vi "Test_C_WS_to_CAN_to_WS.vi"() -> ()   [LabVIEW 2021]
uses:
  CANsub_C.lvlib
  codec_vis/CANsub_Codec.lvlib
  common/Typedefs/Bytes.ctl
  common/CANsub_Common.lvlib
  common/Typedefs/CAN_Frame.ctl
  C_Decode_Result.ctl
panel:
  out "error out":errorcluster
  out "ping payload":u8[](array[numeric]) format="%.0x"
  out "C_Decode_Result":T1={"n frames"=1, "peer close"=FALSE, "ping len"=-1, "crc errors"=0, "decode errors"=0}
  out "frames":T2[](array[typedef])=[{"t_dev"=1735689600.0, "id"=291, "ide"=FALSE, "fdf"=FALSE, "rtr"=FALSE, "brs"=FALSE, "esi"=FALSE, "tx_ack"=FALSE, "error"=FALSE, "err type"=0, "dlc"=3, "data"=[1, 2, 3]}] {"id" format="%.0x"}
  out "ws frame":u8[](array[numeric])=[130, 146, 18, 52, 86, 120, 108, 52, 86, 120, 18, 52, 86, 123, 19, 23, 87, 122, 17, 236, 13, 188, 188, 74] format="%.0x"
  in  "data":u8[](array[numeric])=[1, 2, 3] format="%.0x"
  in  "brs":bool
  in  "fdf":bool
  in  "ide":bool
  in  "id":u32=291 format="%.0x"
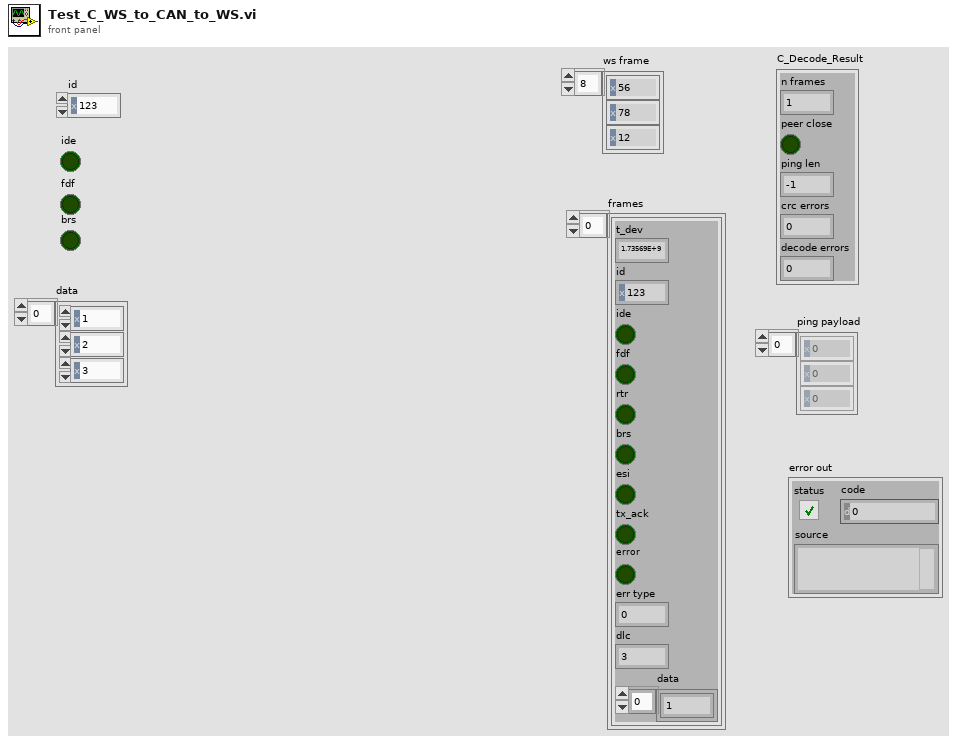
[diagram p1: front panel]
types:
  T1 = typedef "CANsub_C.lvlib/C_Decode_Result.ctl" = cluster{"n frames":i32, "peer close":bool, "ping len":i32, "crc errors":u32, "decode errors":i32}
  T2 = typedef "CANsub_Common.lvlib/CAN_Frame.ctl" = cluster{"t_dev":dbl, "id":u32, "ide":bool, "fdf":bool, "rtr":bool, "brs":bool, "esi":bool, "tx_ack":bool, "error":bool, "err type":u8, "dlc":u8, "data":T3}
  T3 = typedef "CANsub_Common.lvlib/Bytes.ctl" = u8[]
  T4 = typedef "CANsub_C.lvlib/C_State.ctl" = u8[]
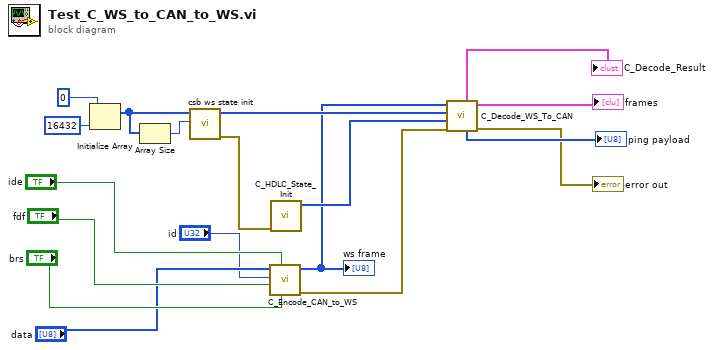
[diagram p0: block diagram]
diagram:
  n1 = Initialize Array(u8 0, 16432 ("dimension size")) -> (w15:u8[])
  n2 = Array Size(array=w15) -> (size(s)=w16:i32)
  n3 = call "csb ws state init.vi"("state_size"=w16, "state"=w15) -> ("error out"=w12:errorcluster, "state_out"=w14:u8[])  [unwired: 7 in, 1 out]
  n4 = call "C_Encode_CAN_to_WS.vi"("brs"="brs", "ide"="ide", "fdf"="fdf", "id"="id", "data"="data") -> ("error out"=w7:errorcluster, "ws frame"=w8:u8[])  [unwired: 5 in]
  "ws frame" <- w8
  n5 = call "C_HDLC_State_Init.vi"("error in (no error)"=w12) -> ("C_State"=w13:T4)  [unwired: 9 in, 1 out]
  n6 = call "C_Decode_WS_To_CAN.vi"("error in (no error)"=w7, "hdlc state in"=w13, "ws state in"=w14, "bytes in"=w8) -> ("error out"=→"error out":errorcluster, "frames"=→"frames":T2[], "ping payload"=→"ping payload":u8[], "result"=→"C_Decode_Result":T1)  [unwired: 2 in, 2 out]
